vi "FuncVI-scat.vi"(5 "InstanceRef":T2, 9 "arg list":T1[](array[typedef]) {"num" format="%.2f"}) -> (0 "error out":bool, 3 "result":T1 {"num" format="%.2f"})   [LabVIEW 2021]
doc: "::: CalcExpress Toolkit :::\nCopyright (c) 2000-2026 Konstantin Shifershteyn. All rights reserved."
uses:
  cetypes.llb/CalcExpress Function Argument Info.ctl
  cetypes.llb/CalcExpress Instance RefNum.ctl
panel:
  in  "max arg num":i32=1000
  in  "min arg num":i32=1
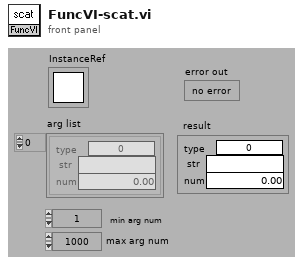
[diagram p1: front panel]
types:
  T1 = typedef "CalcExpress Function Argument Info.ctl" = cluster{"type":u32, "str":string, "num":dbl}
  T2 = typedef "CalcExpress Instance RefNum.ctl" = refnum<k1>
  T3 = enum32{"String", "DBL Number", "identifier", "1D Array of DBL", "2D Array of DBL", "CDB Number", "1D Array of CDB", "2D Array of CDB", "1D Array of String", "2D Array of String", "Unknown data type"}
  T4 = cluster{"type":enum32{"String", "DBL Number", "identifier", "1D Array of DBL", "2D Array of DBL", "CDB Number", "1D Array of CDB", "2D Array of CDB", "1D Array of String", "2D Array of String", "Unknown data type"}, string, "return value":dbl}
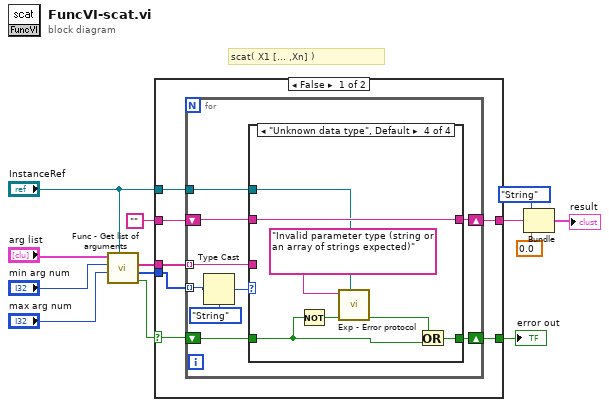
[diagram p0: block diagram]
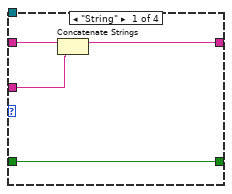
[diagram p2: hidden frame]
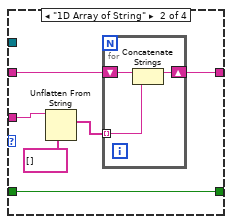
[diagram p3: hidden frame]
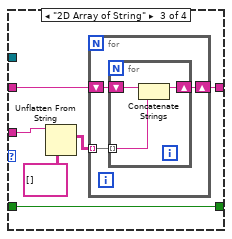
[diagram p4: hidden frame]
diagram:
  # "scat( X1 [... ,Xn] )"
  n1 = call "Func - Get list of arguments.vi"("InstanceRef"="InstanceRef", "max arg num"="max arg num", "min arg num"="min arg num", "arg list"="arg list") -> ("error out"=w6:bool, "type list"=w12:u32[], "str list"=w13:string[])  [unwired: 4 in, 1 out]
  n2 = case shown="False" w6 {
    selector: w6 -> [w16 w62]
    tunnel: w13 -> [w20 _]
    tunnel: w12 -> [w17 _]
    tunnel: "" -> [w19 w63]
    tunnel: [w18 w63] -> w10
    tunnel: "InstanceRef" -> [w15 _]
    tunnel: [w14 w62] -> w3
    frame False {
      n3 = for {
        shift-right: [w27] -> w18
        shift-left: w19 -> [w26]
        tunnel: w20 -> [w29] mode=indexing
        tunnel: w17 -> [w28] mode=indexing
        shift-right: [w24] -> w14
        shift-left: w16 -> [w25]
        tunnel: w15 -> [w23]
        n4 = Type Cast(type=T3."String", x=w28) -> (*(type *) &x=w22:T3)
        n5 = case shown="\"Unknown data type\", Default" w22 {
          tunnel: w29 -> [w32 w39 w48 _]
          tunnel: [w31 w36 w45 w61] -> w27
          tunnel: w26 -> [w33 w35 w44 w61]
          tunnel: w25 -> [w30 w34 w43 w57]
          tunnel: [w30 w34 w43 w59] -> w24
          tunnel: w23 -> [_ _ _ w60]
          frame "String" {
            n6 = Concatenate Strings(w33, w32) -> (w31:string)
          }
          frame "1D Array of String" {
            n7 = Unflatten From String(type=string[] [] ("num list"), binary string=w39) -> (value=w37:string[])  [unwired: 3 in, 2 out]
            n8 = for {
              tunnel: w37 -> [w40] mode=indexing
              shift-right: [w41] -> w36
              shift-left: w35 -> [w42]
              n9 = Concatenate Strings(w42, w40) -> (w41:string)
            }
          }
          frame "2D Array of String" {
            n10 = Unflatten From String(type=string[][] [] ("num list"), binary string=w48) -> (value=w46:string[][])  [unwired: 3 in, 2 out]
            n11 = for {
              tunnel: w46 -> [w51] mode=indexing
              shift-right: [w50] -> w45
              shift-left: w44 -> [w49]
              n12 = for {
                tunnel: w51 -> [w52] mode=indexing
                shift-right: [w53] -> w50
                shift-left: w49 -> [w54]
                n13 = Concatenate Strings(w54, w52) -> (w53:string)
              }
            }
          }
          frame "Unknown data type", Default {
            n14 = Not(x=w57) -> (.not. x?=w56:bool)
            n15 = call "Exp - Error protocol.vi"("InstanceRef"=w60, "error in"=w56, "error message in"="Invalid parameter type (string or an array of strings expected)" ("ErrStr")) -> ("error out"=w58:bool)  [unwired: 5 in, 1 out]
            n16 = Or(x=w58, y=w57) -> (x .or. y?=w59:bool)
          }
        }
      }
    }
    frame True {
    }
  }
  "error out" <- w3
  n17 = Bundle("type"=T3."String", w10, "return value"=0.0) -> (→"result":T4)  [unwired: 1 in]
